vi "CSE - Parse Script.vi"(5 "directives":T1={"enaNamedConst"=TRUE}, 6 "parameters":T2={"AutoParse"=TRUE, "GroupStm"=FALSE, "ErrSrcMaxLen"=180}, 7 "Script name":string, 8 "error in":errorcluster, 9 "action":u32(ring) items=["parse", "parse (dyn instance)", "test syntax"], 10 "load FuncVIs":u32(ring)=2 items=["don't load", "load", "load & test"], 11 "Script":string) -> (0 "error out":errorcluster, 1 "dynamic instance":bool, 2 "loaded functions":string[](array[string]), 3 "CSE RefNum":T3, 4 "parsed":bool)   [LabVIEW 2021]
doc: "This VI parses a CSE script. Refer to the VI help for more details.\n\n<b>Script</b> specifies the CSE script to be parsed.\n\n<b>action</b> control specifies the operation to perform:\n 'parse' : parses a script and saves the parsed script in the static context of the current VI instance.\n 'parse (dyn instance)' : creates a new dynamic CSE instance context and saves the parsed script in it. A dynamic CSE instance context must be explicitly closed.\n 'test syntax' : identical to the 'parse' action, except the VI closes references to FuncVIs after parsing.\n\n<b>Script name</b> is an optional parameter. If you specify a name, it is used in error messages along with the line number. This is convenient for identifying an error location when a script calls other scripts.\n\n<b>load FuncVIs</b> control specifies how this VI maintains calls to FuncVI functions found during parsing:\n 'don't load' : does not load FuncVIs.\n 'load' : loads FuncVIs.\n 'load & test' : loads FuncVIs and verifies the correct number of arguments in the function calls.\n\n<b>parameters</b> control is the cluster with the following options:\n <b>AutoParse</b> : if FALSE, the VI parses the script every time it is called. If TRUE (default), the VI parses an input script only if it has not been parsed yet. Enabling this option can significantly decrease execution time if you parse and execute a script in a loop. Note that the VI always parses a script when it creates a dynamic instance context.\n <b>GroupStm</b> : if TRUE, the VI groups a sequence of expression statements into a single statement. This can slightly increase the speed of script execution. The default value is FALSE.\n <b>ErrSrcMaxLen</b> : specifies the maximum length of the source code quotation included in error messages.\n\n<b>CSE RefNum</b> indicator returns a reference to a CSE instance context containing the parsed script.\n\n<b>dynamic instance</b> indicator returns TRUE if a dynamic CSE instance context has been created.\n\n<b>parsed</b> indicator returns TRUE if an input script was actually parsed. It returns FALSE when the static context already contains a parsed version of the input script.\n\n::: CalcExpress Toolkit :::\nCopyright (c) 2000-2026 Konstantin Shifershteyn. All rights reserved."
uses:
  CSE Instance RefNum.ctl
  cetypes.llb/CSE Parsing Options.ctl
  cetypes.llb/CSE Parsing Directives.ctl
  cersrc/celveng32.dll
panel:
  in  "CSE RefNum Tmpl":T3
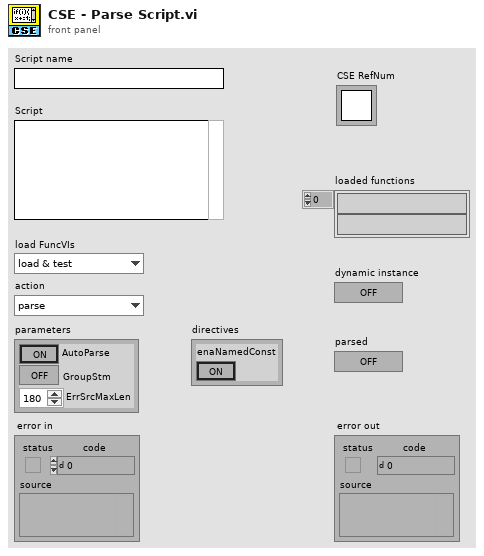
[diagram p1: front panel]
types:
  T1 = typedef "CSE Parsing Directives.ctl" = cluster{"enaNamedConst":bool}
  T2 = typedef "CSE Parsing Options.ctl" = cluster{"AutoParse":bool, "GroupStm":bool, "ErrSrcMaxLen":i32}
  T3 = typedef "CSE Instance RefNum.ctl" = refnum<k1>
  T4 = cluster{"AutoParse":bool, "GroupStm":bool, "ErrSrcMaxLen":i32, "enaNamedConst":bool}
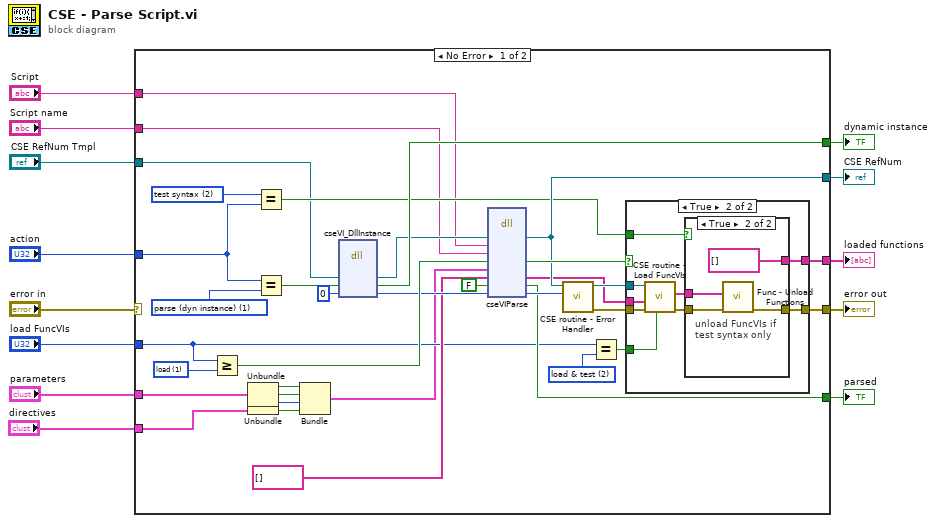
[diagram p0: block diagram]
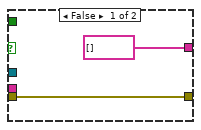
[diagram p2: hidden frame]
diagram:
  n1 = case shown="No Error" "error in" {
    selector: "error in" -> [_ w66]
    tunnel: [w47 w66] -> w10
    tunnel: [w38 _] -> w13
    tunnel: [w42 _] -> w12
    tunnel: [w46 _] -> w11
    tunnel: [w33 _] -> w9
    tunnel: "load FuncVIs" -> [w25 _]
    tunnel: "action" -> [w24 _]
    tunnel: "CSE RefNum Tmpl" -> [w23 _]
    tunnel: "Script name" -> [w22 _]
    tunnel: "Script" -> [w21 _]
    tunnel: "parameters" -> [w20 _]
    tunnel: "directives" -> [w16 _]
    frame No Error {
      w29 = u32 2 items=["parse", "parse (dyn instance)", "test syntax"] ("action")
      w30 = u32 1 items=["parse", "parse (dyn instance)", "test syntax"] ("action")
      w44 = u32 2 items=["don't load", "load", "load & test"] ("load FuncVIs")
      w45 = u32 1 items=["don't load", "load", "load & test"] ("load FuncVIs")
      n2 = Greater Or Equal?(x=w25, y=w45) -> (x >= y?=w41:bool)
      n3 = Unbundle(w20) -> ("AutoParse"=w19:bool, "GroupStm"=w18:bool, "ErrSrcMaxLen"=w17:i32)
      n4 = Unbundle(w16) -> ("enaNamedConst"=w14:bool)
      n5 = Equal?(x=w29, y=w24) -> (x = y?=w28:bool)
      n6 = Equal?(x=w24, y=w30) -> (x = y?=w31:bool)
      n7 = Bundle("AutoParse"=w19, "GroupStm"=w18, "ErrSrcMaxLen"=w17, "enaNamedConst"=w14) -> (w15:T4)  [unwired: 1 in]
      n8 = dll-call lib="C:/LV Projects/CalcExpress 40 LV2021/vi.lib/addons/CalcExpress/cersrc/celveng*.dll" fn="cseVI_DllInstance"("iRef"=w23, "newInst"=w31, "erStat"=0) -> ("iRef"=w26:T3, "newInst"=w42:bool, "erStat"=w36:i32)  [unwired: 6 in, 2 out]
      n9 = dll-call lib="C:/LV Projects/CalcExpress 40 LV2021/vi.lib/addons/CalcExpress/cersrc/celveng*.dll" fn="cseVIParse" ("viCESPParse")("iRef"=w26, "script"=w21, "scriptName"=w22, "fFVI"=w41, "params"=w15, "aFVI"=string[] [], "fParsed"=FALSE ("performed"), "erStat"=w36) -> ("iRef"=w38:T3, "fFVI"=w40:bool, "aFVI"=w34:string[], "fParsed"=w33:bool, "erStat"=w37:i32)  [unwired: 7 in, 2 out]
      n10 = call "CSE routine - Error Handler.vi"("exec status"=w37, "CSE RefNum"=w38) -> ("error out"=w48:errorcluster, "dup CSE RefNum"=w39:T3)  [unwired: 5 in, 1 out]
      n11 = Equal?(x=w25, y=w44) -> (x = y?=w43:bool)
      n12 = case shown="True" w40 {
        tunnel: w48 -> [w50 w59]
        tunnel: w34 -> [_ w58]
        tunnel: [w50 w56] -> w47
        tunnel: [string[] [] ("loaded functions") w54] -> w46
        tunnel: w43 -> [_ w53]
        tunnel: w39 -> [_ w52]
        tunnel: w28 -> [_ w51]
        frame False {
        }
        frame True {
          n13 = call "CSE routine - Load FuncVIs.vi"("test arg num"=w53, "error in"=w59, "FuncVIs info"=w58, "CSE RefNum"=w52) -> ("error out"=w57:errorcluster, "loaded functions"=w55:string[])  [unwired: 4 in]
          n14 = case shown="True" w51 {
            tunnel: [w61 w63] -> w56
            tunnel: w57 -> [w61 w65]
            tunnel: [w60 string[] []] -> w54
            tunnel: w55 -> [w60 w64]
            frame False {
            }
            frame True {
              # "unload FuncVIs if test syntax only"
              n15 = call "Func - Unload Functions.vi"("error in"=w65, "Array of func names"=w64) -> ("error out"=w63:errorcluster)  [unwired: 7 in]
            }
          }
        }
      }
    }
    frame Error {
    }
  }
  "error out" <- w10
  "CSE RefNum" <- w13
  "dynamic instance" <- w12
  "loaded functions" <- w11
  "parsed" <- w9
